vi "Envoi alarmes MODBUS EPC.vi"(3 "Alarme haute":dbl, 4 "Alarme basse":dbl, 5 "Fichier de rapport":path) -> ()   [LabVIEW 2022 SP3]
uses:
  Variables globales/Variables glob EUROTHERM.vi
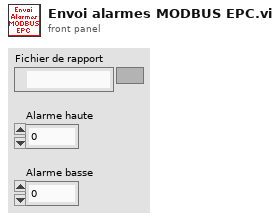
[diagram p1: front panel]
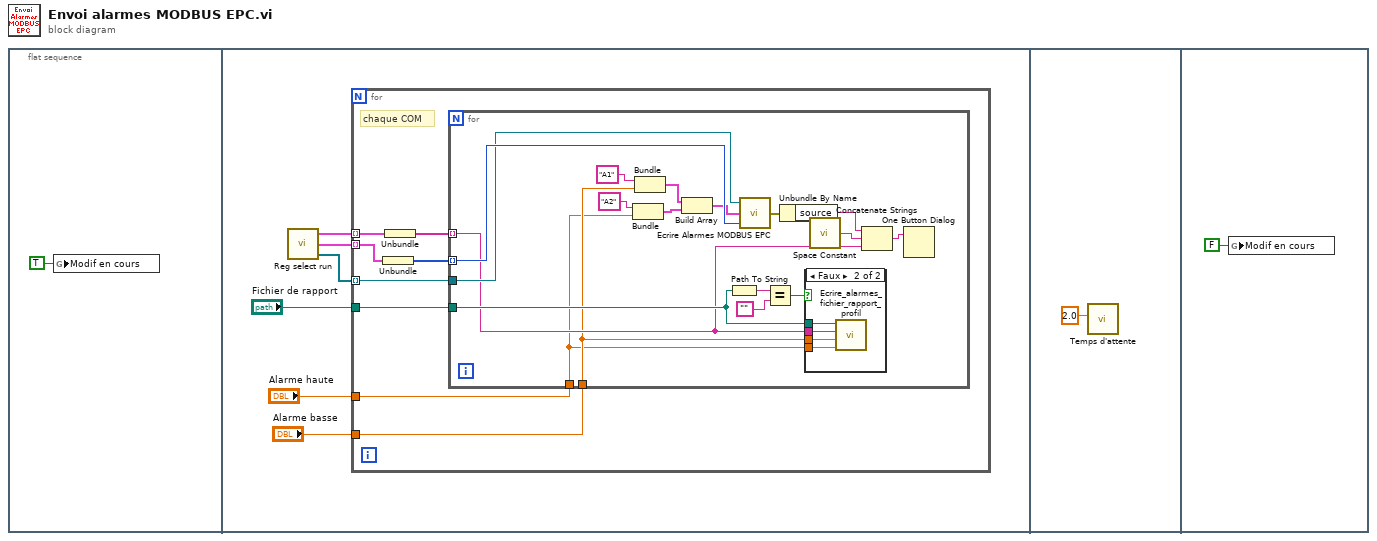
[diagram p0: block diagram]
diagram:
  n1 = flat-sequence {
    frame #0 {
      n2 = global write "Variables glob EUROTHERM.vi" "Modif en cours"(TRUE ("Modif en cours")) -> ()
    }
    frame #1 {
      n3 = call "Reg select run.vi"() -> ("Noms sélect run"=w5:cluster{"Noms voies sélect run 1COM":string[]}[], "Adresses sélect run"=w6:cluster{"Adresses run 1COM reg":u8[]}[], "COM run"=w2:refnum<visa-resource-name>[])  [unwired: 2 in]
      n4 = for {
        tunnel: w5 -> [w15] mode=indexing
        tunnel: w6 -> [w13] mode=indexing
        tunnel: "Alarme basse" -> [w11]
        tunnel: "Alarme haute" -> [w10]
        tunnel: "Fichier de rapport" -> [w9]
        tunnel: w2 -> [w8] mode=indexing
        # "chaque COM"
        n5 = Unbundle(w13) -> ("Adresses run 1COM reg"=w12:u8[])
        n6 = Unbundle(w15) -> ("Noms voies sélect run 1COM"=w14:string[])
        n7 = for {
          tunnel: w14 -> [w20] mode=indexing
          tunnel: w12 -> [w33] mode=indexing
          tunnel: w8 -> [w32]
          tunnel: w11 -> [w17]
          tunnel: w10 -> [w16]
          tunnel: w9 -> [w23]
          n8 = Bundle("A2", "Alarme haute"=w16) -> (w18:cluster{string, "Alarme haute":dbl})  [unwired: 1 in]
          n9 = Bundle("A1", "Alarme basse"=w17) -> (w30:cluster{string, "Alarme basse":dbl})  [unwired: 1 in]
          n10 = Build Array(w30, w18) -> (w31:cluster{string, "Alarme haute":dbl}[])
          n11 = Path To String(path=w23) -> (string=w27:string)
          n12 = call "Ecrire Alarmes MODBUS EPC.vi"("Adresse rég"=w33, "Programmation configuration"=w31, "Port COM run 1 REG"=w32) -> ("error out"=w24:errorcluster)
          n13 = Equal?(x=w27, y="") -> (x = y?=w25:bool)
          n14 = Unbundle By Name(w24) -> ("source"=w22:string)
          n15 = case shown="Faux" w25 {
            tunnel: w17 -> [_ w37]
            tunnel: w16 -> [_ w36]
            tunnel: w20 -> [_ w35]
            tunnel: w23 -> [_ w34]
            frame True {
            }
            frame False {
              n16 = call "Ecrire_alarmes_fichier_rapport_profil.vi"("Alarme haute (°C)"=w36, "Alarme basse (°C)"=w37, "Nom Regulateur"=w35, "Fichier rapport"=w34) -> ()  [unwired: 1 in]
            }
          }
          n17 = call <vilib>:"Space Constant.vi"() -> ("String"=w19:string)
          n18 = Concatenate Strings(w22, w19, w20) -> (w21:string)
          n19 = One Button Dialog(message=w21) -> ()  [unwired: 1 in, 1 out]
        }
      }
    }
    frame #2 {
      n20 = call "Temps d'attente"("Delay Time (s)"=2.0) -> ()  [unwired: 10 in, 1 out]
    }
    frame #3 {
      n21 = global write "Variables glob EUROTHERM.vi" "Modif en cours"(FALSE ("Modif en cours")) -> ()
    }
  }
